vi "init 3D Controller.vi"(8 "error in (no error)":errorcluster, 10 "VISA resource name":refnum<visa-resource-name>, 11 "3D Controller in":refnum<class "3D Controller.lvclass">) -> (0 "error out":errorcluster, 2 "Connected?":bool, 3 "3D Controller out":refnum<class "3D Controller.lvclass">)   [LabVIEW 2023, in "FCC 3D Controller for BS.lvlib" / "3D Controller.lvclass"]
uses:
  3D Controller.lvclass
  Type Definition/TYPE Serial Port Setting.ctl
  Type Definition/TYPE Protocol Char of Command.ctl
  3D Controller.lvclass/3D Controller.ctl
  FCC 3D Controller for BS.lvlib
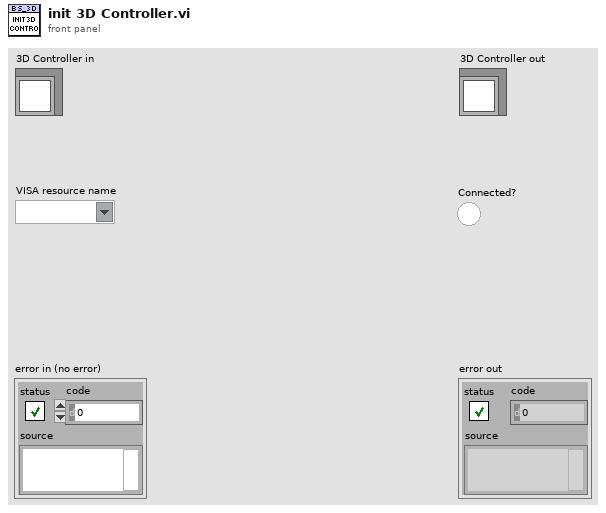
[diagram p1: front panel]
types:
  T1 = typedef "FCC 3D Controller for BS.lvlib/TYPE Protocol Char of Command.ctl" = cluster{"Header":string, "Axis No.":i32, "End":string}
  T2 = typedef "FCC 3D Controller for BS.lvlib/TYPE Serial Port Setting.ctl" = cluster{"Baud Rate":u32, "Termination Character":u8, "Termination Character Enable":bool, "Flush I/O Buffer mask":u16}
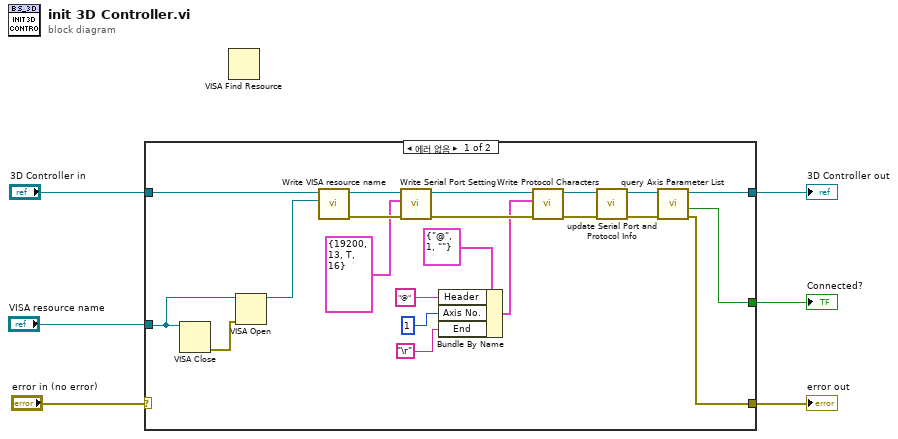
[diagram p0: block diagram]
diagram:
  n1 = case shown="에러 없음" "error in (no error)" {
    selector: "error in (no error)" -> [_ w28]
    tunnel: "3D Controller in" -> [w27 w29]
    tunnel: [w12 w29] -> w4
    tunnel: [w11 w28] -> w3
    tunnel: "VISA resource name" -> [w9 _]
    tunnel: [w10 _] -> w1
    frame No Error {
      n2 = VISA Close(VISA resource name=w9) -> (error out=w8:errorcluster)  [unwired: 1 in]
      n3 = VISA Open(error in (no error)=w8, VISA resource name=w9) -> (VISA resource name=w7:refnum<visa-resource-name>)  [unwired: 3 in, 1 out]
      n4 = call "Write VISA resource name.vi"("VISA resource name"=w7, "3D Controller in"=w27) -> ("error out"=w25:errorcluster, "3D Controller out"=w26:refnum<class "3D Controller.lvclass">)  [unwired: 8 in]
      n5 = call "Write Serial Port Setting.vi"("error in (no error)"=w25, "Serial Port Setting"=T2 {"Baud Rate"=19200, "Termination Character"=13, "Termination Character Enable"=TRUE, "Flush I/O Buffer mask"=16}, "3D Controller in"=w26) -> ("error out"=w22:errorcluster, "3D Controller out"=w23:refnum<class "3D Controller.lvclass">)  [unwired: 7 in]
      n6 = Bundle By Name(cluster=T1 {"Header"="@", "Axis No."=1, "End"=""} ("Protocol Characters"), "Header"="@", "Axis No."=1, "End"="\r") -> (w19:T1)
      n7 = call "Write Protocol Characters.vi"("error in (no error)"=w22, "Protocol Characters"=w19, "3D Controller in"=w23) -> ("error out"=w17:errorcluster, "3D Controller out"=w18:refnum<class "3D Controller.lvclass">)  [unwired: 7 in]
      n8 = call "update Serial Port and Protocol Info.vi"("error in (no error)"=w17, "3D Controller in"=w18) -> ("error out"=w13:errorcluster, "3D Controller out"=w14:refnum<class "3D Controller.lvclass">)  [unwired: 8 in]
      n9 = call-dynamic "query Axis Parameter List.vi"("error in (no error)"=w13, "3D Controller in"=w14) -> ("error out"=w11:errorcluster, "Valid"=w10:bool, "3D Controller out"=w12:refnum<class "3D Controller.lvclass">)  [unwired: 6 in, 1 out]
    }
    frame Error {
    }
  }
  "error out" <- w3
  "3D Controller out" <- w4
  "Connected?" <- w1
  n10 = VISA Find Resource() -> ()  [unwired: 3 in, 3 out]
